vi "LCP table array ans.vi"(6 "LSP Table":string[][](table) caption="LS Table", 8 "error in (no error)":errorcluster caption="error in", 9 "LAP Table":string[][](table), 10 "LCP Table":string[][](table) caption="CP Table", 11 "Tag cluster_B":T3) -> (0 "error out":errorcluster, 1 "LSPX_C2":T4, 2 "LSPX_C1":T5, 3 "LCPX_C1":T6, 5 "LCPX_CZ":T1)   [LabVIEW 2018]
panel:
  out "LCPX_C2":T2
  out "LA_Signal Intensity [pA]":dbl[](array[numeric])
  out "MS_IDX":i32[](array[numeric])
  out "LA_Time":dbl[](array[numeric])
  out "LA_Relative Averaged Data":dbl[](array[numeric])
  out "LAP Table Tag":string[](array[string])
  out "Signal Intensity [pA]":dbl[](array[numeric])
  out "Base Number":i32[](array[numeric])
  out "L#":i32[](array[numeric])
  out "Signal Intensity [pA]":string[](array[string])
  out "Base Number":string[](array[string])
  out "Mx Right Read Seq":string[](array[string])
  out "L#":string[](array[string])
  out "Assinged Sequence":string[](array[string])
  out "Signal End [s]":dbl[](array[numeric])
  out "Signal Start [s]":dbl[](array[numeric])
  out "S IDX":i32[](array[numeric])
  out "Mx Right No":i32[](array[numeric])
  out "Seq ENo":i32[](array[numeric])
  out "Seq SNo":i32[](array[numeric])
  out "Signal End [s]":string[](array[string])
  out "S IDX":string[](array[string])
  out "Signal Start [s]":string[](array[string])
  out "Direction":string[](array[string])
  out "Seq ENo":string[](array[string])
  out "Mx Right No":string[](array[string])
  out "Seq SNo":string[](array[string])
  out "5’→3'":bool[](array[boolean])
  out "5’→3'":dbl
  out "Signal Length [ms]":dbl[](array[numeric])
  out "Q value [x]":dbl[](array[numeric])
  out "Signal Intensity [pA]":dbl[](array[numeric])
  out "AS IDX":i32[](array[numeric])
  out "Time":dbl[](array[numeric])
  out "Relative Averaged Data":dbl[](array[numeric])
  out "LCP Table Tag":string[](array[string])
  out "LSP Table Tag":string[](array[string])
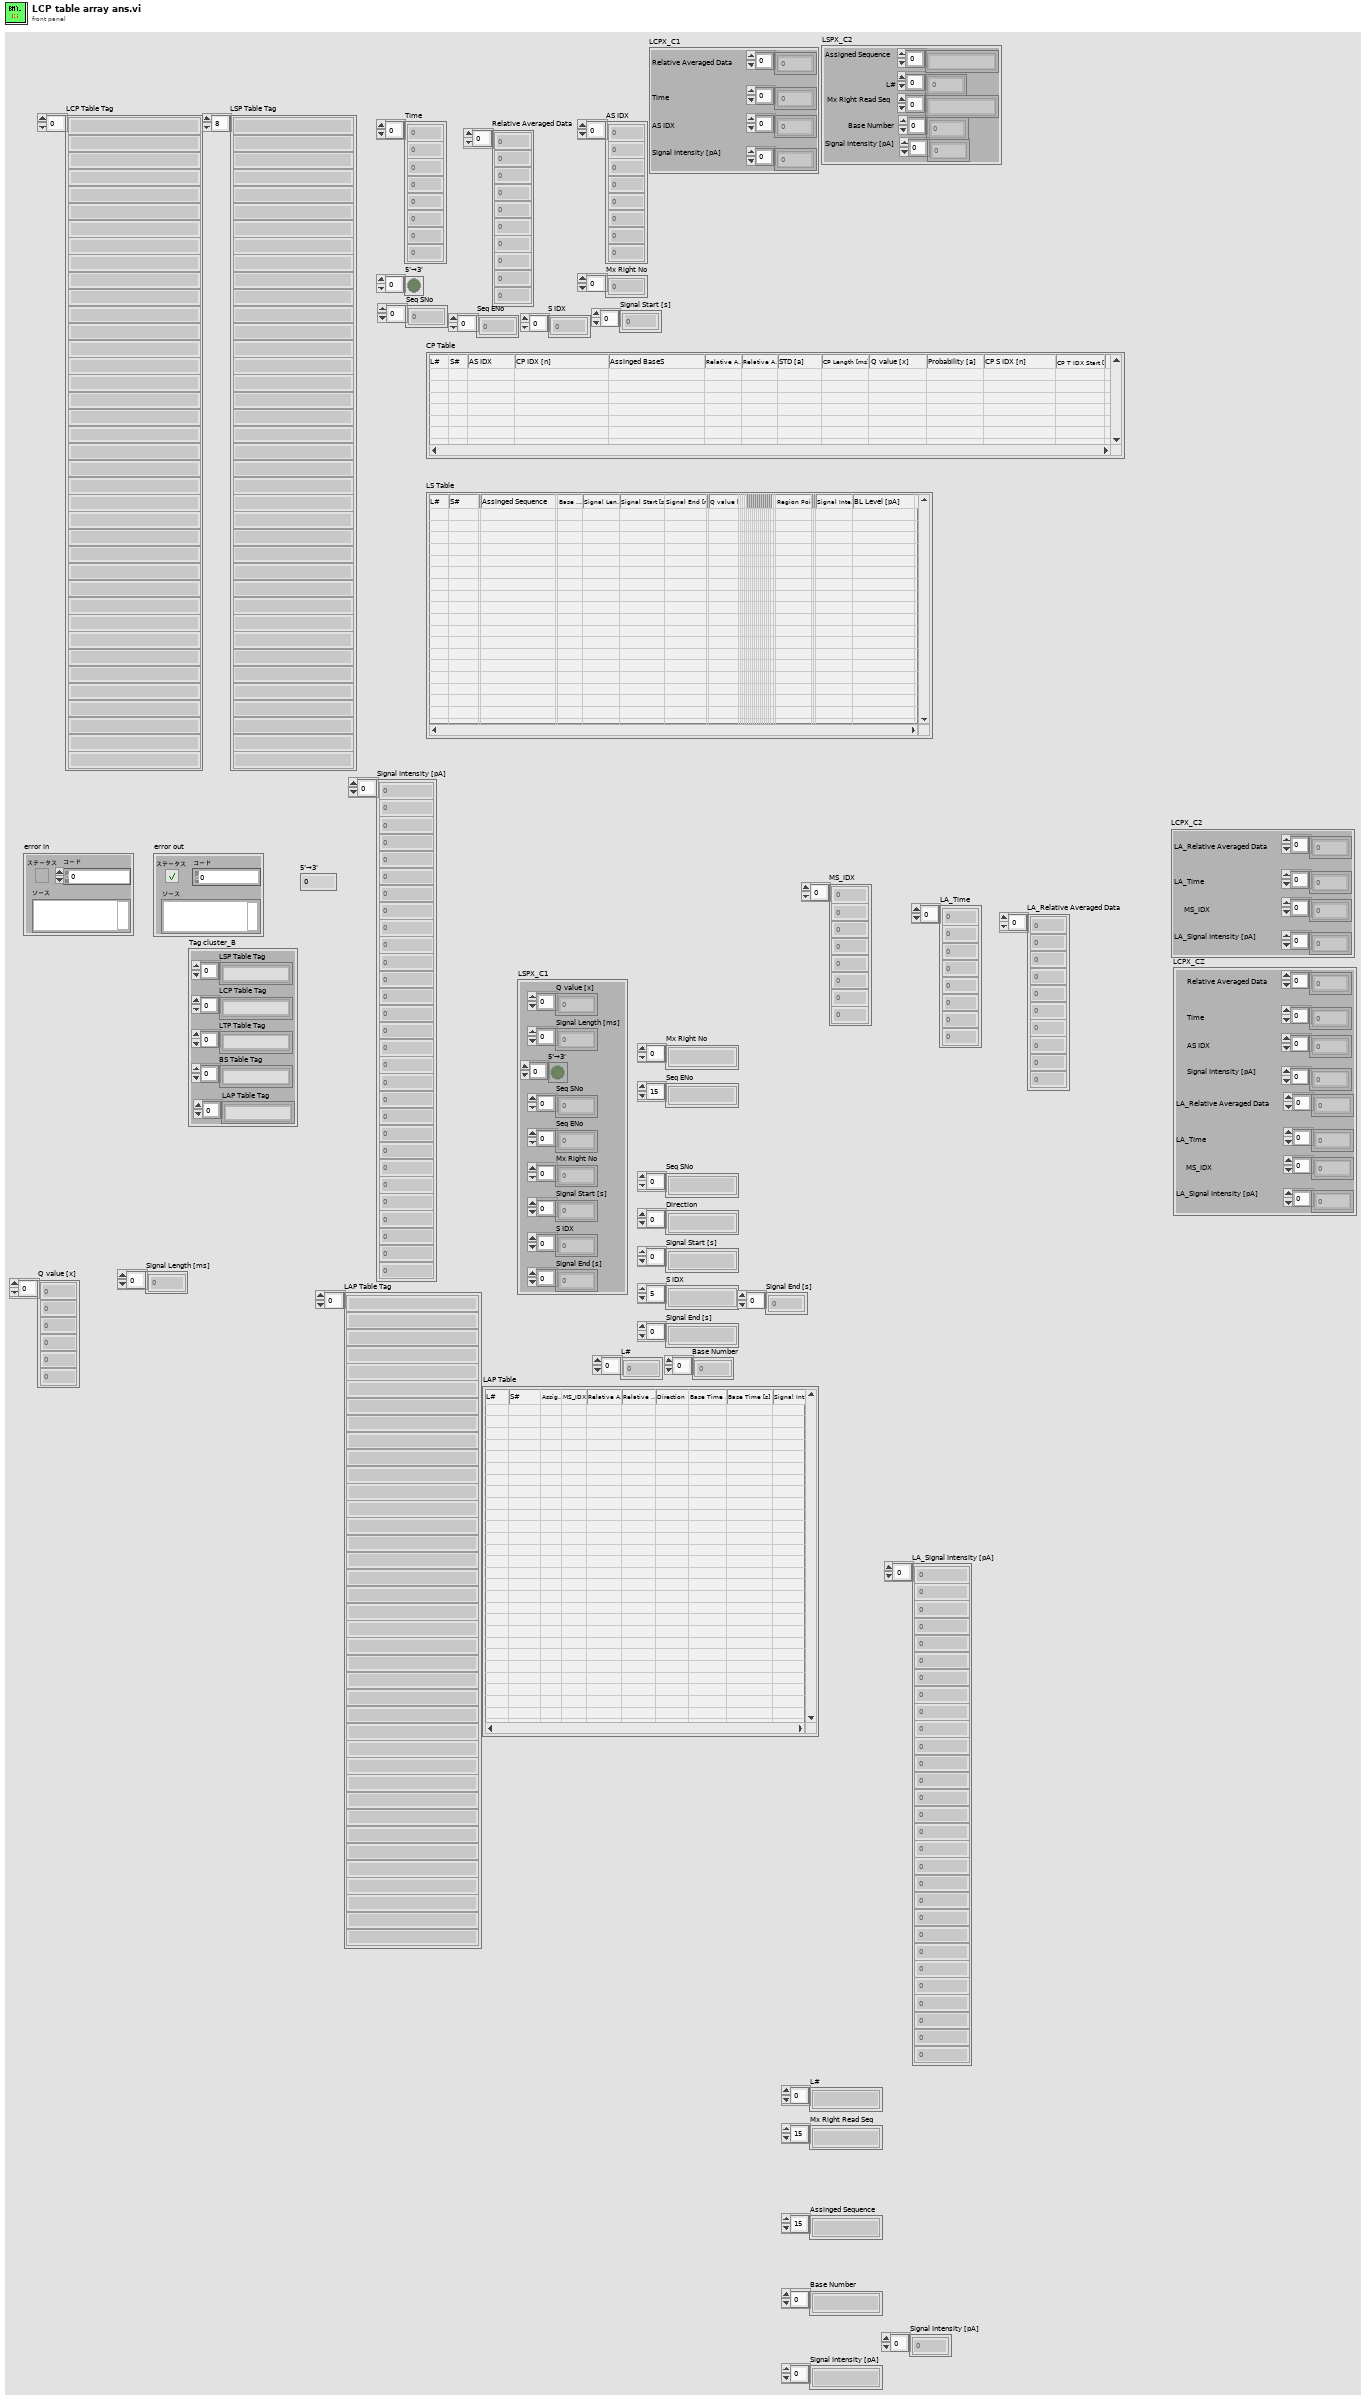
[diagram p1: front panel]
types:
  T1 = cluster{"Relative Averaged Data":dbl[], "Time":dbl[], "AS IDX":i32[], "Signal Intensity [pA]":dbl[], "LA_Relative Averaged Data":dbl[], "LA_Time":dbl[], "MS_IDX":i32[], "LA_Signal Intensity [pA]":dbl[]}
  T2 = cluster{"LA_Relative Averaged Data":dbl[], "LA_Time":dbl[], "MS_IDX":i32[], "LA_Signal Intensity [pA]":dbl[]}
  T3 = cluster{"LSP Table Tag":string[], "LCP Table Tag":string[], "LTP Table Tag":string[], "BS Table Tag":string[], "LAP Table Tag":string[]}
  T4 = cluster{"Assigned Sequence":string[], "L#":i32[], "Mx Right Read Seq":string[], "Base Number":i32[], "Signal Intensity [pA]":dbl[]}
  T5 = cluster{"Q value [x]":dbl[], "Signal Length [ms]":dbl[], "5’→3'":bool[], "Seq SNo":i32[], "Seq ENo":i32[], "Mx Right No":i32[], "Signal Start [s]":dbl[], "S IDX":i32[], "Signal End [s]":dbl[]}
  T6 = cluster{"Relative Averaged Data":dbl[], "Time":dbl[], "AS IDX":i32[], "Signal Intensity [pA]":dbl[]}
  T7 = cluster{dbl[], dbl[], i32[], dbl[], dbl[], dbl[], i32[], dbl[]}
  T8 = cluster{dbl[], dbl[], bool[], i32[], i32[], i32[], dbl[], i32[], dbl[]}
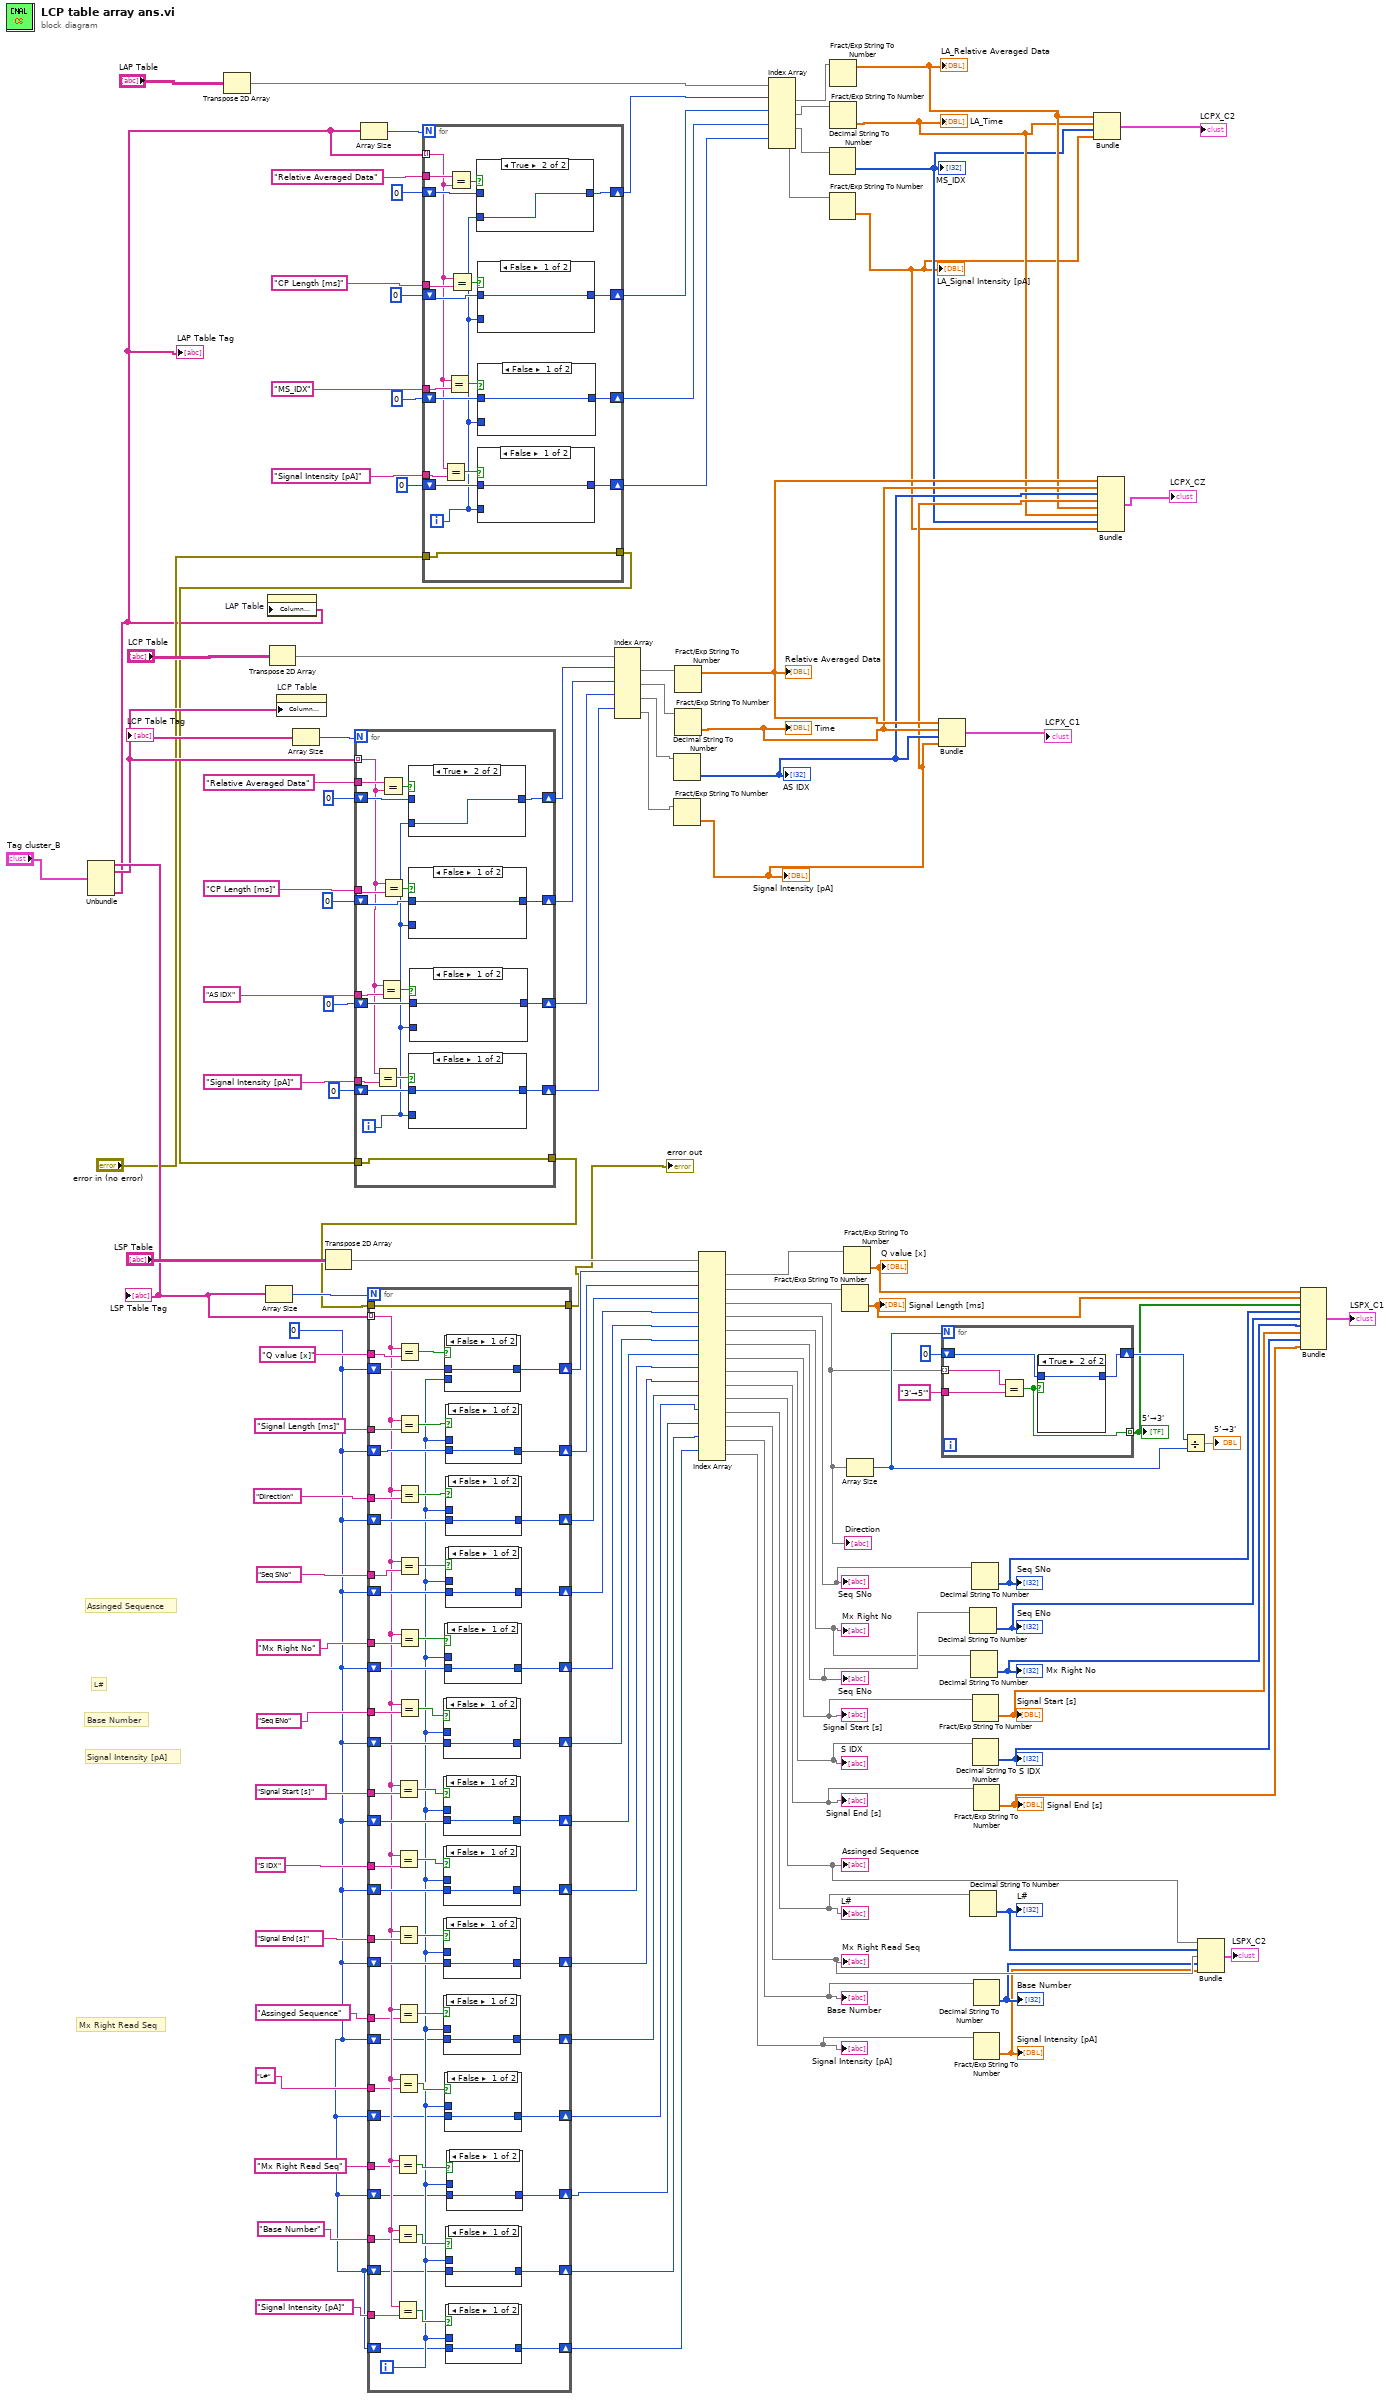
[diagram p0: block diagram]
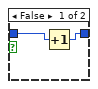
[diagram p6: hidden frame]
diagram:
  w55 = 0
  # "Mx Right Read Seq"
  # "Signal Intensity [pA]"
  # "Base Number"
  # "Assinged Sequence"
  # "L#"
  n1 = Unbundle("Tag cluster_B") -> ("LSP Table Tag"=w34:string[], "LCP Table Tag"=w33:string[], "LAP Table Tag"=w15:string[])  [unwired: 2 out]
  "LSP Table Tag" <- w34
  "LCP Table Tag" <- w33
  "LAP Table Tag" <- w15
  n2 = Transpose 2D Array(2D array="LAP Table") -> (transposed array=w20:string[][])
  n3 = Array Size(array=w34) -> (size(s)=w106:i32)
  n4 = property on="LAP Table" class="Tbl (strict)"("Column Headers[]"=w15) -> ()  [unwired: 2 in, 2 out]
  n5 = Transpose 2D Array(2D array="LCP Table") -> (transposed array=w113:string[][])
  n6 = property on="LCP Table" class="Tbl (strict)"("Column Headers[]"=w33) -> ()  [unwired: 2 in, 2 out]
  n7 = Array Size(array=w33) -> (size(s)=w108:i32)
  n8 = Transpose 2D Array(2D array="LSP Table") -> (transposed array=w101:string[][])
  n9 = Array Size(array=w15) -> (size(s)=w24:i32)
  n10 = for {
    N: w24 -> [_]
    tunnel: "Relative Averaged Data" -> [w141]
    tunnel: w15 -> [w126] mode=indexing
    shift-right: [w139] -> w19
    shift-left: 0 -> [w138]
    tunnel: "CP Length [ms]" -> [w137]
    shift-right: [w135] -> w18
    shift-left: 0 -> [w134]
    shift-right: [w132] -> w17
    shift-left: 0 -> [w131]
    tunnel: "MS_IDX" -> [w130]
    shift-right: [w129] -> w16
    shift-left: 0 -> [w128]
    tunnel: "Signal Intensity [pA]" -> [w125]
    tunnel: "error in (no error)" -> [w124]
    tunnel: [w124] -> w22
    i -> [w123]
    n11 = Equal?(x=w126, y=w125) -> (x = y?=w127:bool)
    n12 = Equal?(x=w126, y=w130) -> (x = y?=w133:bool)
    n13 = Equal?(x=w141, y=w126) -> (x = y?=w140:bool)
    n14 = Equal?(x=w126, y=w137) -> (x = y?=w136:bool)
    n15 = case shown="True" w140 {
      tunnel: w123 -> [_ w149]
      tunnel: [w148 w149] -> w139
      tunnel: w138 -> [w148 _]
      frame False {
      }
      frame True {
      }
    }
    n16 = case shown="False" w136 {
      tunnel: w123 -> [_ w147]
      tunnel: [w146 w147] -> w135
      tunnel: w134 -> [w146 _]
      frame False {
      }
      frame True {
      }
    }
    n17 = case shown="False" w127 {
      tunnel: w123 -> [_ w143]
      tunnel: [w142 w143] -> w129
      tunnel: w128 -> [w142 _]
      frame False {
      }
      frame True {
      }
    }
    n18 = case shown="False" w133 {
      tunnel: w123 -> [_ w145]
      tunnel: [w144 w145] -> w132
      tunnel: w131 -> [w144 _]
      frame False {
      }
      frame True {
      }
    }
  }
  n19 = for {
    N: w108 -> [_]
    tunnel: "Relative Averaged Data" -> [w168]
    tunnel: w33 -> [w153] mode=indexing
    shift-right: [w166] -> w39
    shift-left: 0 -> [w165]
    tunnel: "CP Length [ms]" -> [w164]
    shift-right: [w162] -> w38
    shift-left: 0 -> [w161]
    shift-right: [w159] -> w110
    shift-left: 0 -> [w158]
    tunnel: "AS IDX" -> [w157]
    shift-right: [w156] -> w37
    shift-left: 0 -> [w155]
    tunnel: "Signal Intensity [pA]" -> [w152]
    tunnel: w22 -> [w151]
    tunnel: [w151] -> w62
    i -> [w150]
    n20 = Equal?(x=w153, y=w152) -> (x = y?=w154:bool)
    n21 = Equal?(x=w153, y=w157) -> (x = y?=w160:bool)
    n22 = Equal?(x=w168, y=w153) -> (x = y?=w167:bool)
    n23 = Equal?(x=w153, y=w164) -> (x = y?=w163:bool)
    n24 = case shown="True" w167 {
      tunnel: w150 -> [_ w176]
      tunnel: [w175 w176] -> w166
      tunnel: w165 -> [w175 _]
      frame False {
      }
      frame True {
      }
    }
    n25 = case shown="False" w163 {
      tunnel: w150 -> [_ w174]
      tunnel: [w173 w174] -> w162
      tunnel: w161 -> [w173 _]
      frame False {
      }
      frame True {
      }
    }
    n26 = case shown="False" w154 {
      tunnel: w150 -> [_ w170]
      tunnel: [w169 w170] -> w156
      tunnel: w155 -> [w169 _]
      frame False {
      }
      frame True {
      }
    }
    n27 = case shown="False" w160 {
      tunnel: w150 -> [_ w172]
      tunnel: [w171 w172] -> w159
      tunnel: w158 -> [w171 _]
      frame False {
      }
      frame True {
      }
    }
  }
  n28 = for {
    N: w106 -> [_]
    tunnel: w34 -> [w198] mode=indexing
    tunnel: "Q value [x]" -> [w235]
    tunnel: "Signal Length [ms]" -> [w234]
    tunnel: "Direction" -> [w233]
    shift-right: [w229] -> w102
    shift-left: w55 -> [w228]
    shift-right: [w227] -> w99
    shift-left: w55 -> [w226]
    shift-right: [w225] -> w97
    shift-left: w55 -> [w224]
    tunnel: "Seq SNo" -> [w223]
    tunnel: "Mx Right No" -> [w222]
    tunnel: "Seq ENo" -> [w221]
    tunnel: "Signal Start [s]" -> [w220]
    tunnel: "S IDX" -> [w219]
    tunnel: "Signal End [s]" -> [w218]
    shift-right: [w211] -> w84
    shift-left: w55 -> [w210]
    shift-right: [w209] -> w83
    shift-left: w55 -> [w208]
    shift-right: [w207] -> w82
    shift-left: w55 -> [w206]
    shift-right: [w205] -> w80
    shift-left: w55 -> [w204]
    shift-right: [w203] -> w79
    shift-left: w55 -> [w202]
    shift-right: [w201] -> w78
    shift-left: w55 -> [w200]
    tunnel: w62 -> [w199]
    tunnel: [w199] -> w61
    tunnel: "Base Number" -> [w197]
    tunnel: "Signal Intensity [pA]" -> [w192]
    tunnel: "Assinged Sequence" -> [w190]
    tunnel: "L#" -> [w189]
    shift-right: [w188] -> w54
    shift-left: w55 -> [w186]
    shift-right: [w185] -> w53
    shift-left: w55 -> [w184]
    shift-right: [w183] -> w51
    shift-left: w55 -> [w182]
    shift-right: [w181] -> w50
    shift-left: w55 -> [w180]
    shift-right: [w179] -> w49
    shift-left: w55 -> [w178]
    tunnel: "Mx Right Read Seq" -> [w177]
    i -> [w187]
    n29 = Equal?(x=w198, y=w177) -> (x = y?=w194:bool)
    n30 = Equal?(x=w198, y=w197) -> (x = y?=w193:bool)
    n31 = Equal?(x=w198, y=w192) -> (x = y?=w191:bool)
    n32 = Equal?(x=w198, y=w220) -> (x = y?=w214:bool)
    n33 = Equal?(x=w198, y=w219) -> (x = y?=w213:bool)
    n34 = Equal?(x=w198, y=w218) -> (x = y?=w212:bool)
    n35 = Equal?(x=w198, y=w190) -> (x = y?=w196:bool)
    n36 = Equal?(x=w198, y=w189) -> (x = y?=w195:bool)
    n37 = Equal?(x=w198, y=w235) -> (x = y?=w232:bool)
    n38 = Equal?(x=w198, y=w234) -> (x = y?=w231:bool)
    n39 = Equal?(x=w198, y=w233) -> (x = y?=w230:bool)
    n40 = Equal?(x=w198, y=w223) -> (x = y?=w217:bool)
    n41 = Equal?(x=w198, y=w222) -> (x = y?=w216:bool)
    n42 = Equal?(x=w198, y=w221) -> (x = y?=w215:bool)
    n43 = case shown="False" w215 {
      tunnel: w187 -> [_ w253]
      tunnel: [w252 w253] -> w207
      tunnel: w206 -> [w252 _]
      frame False {
      }
      frame True {
      }
    }
    n44 = case shown="False" w214 {
      tunnel: w187 -> [_ w251]
      tunnel: [w250 w251] -> w205
      tunnel: w204 -> [w250 _]
      frame False {
      }
      frame True {
      }
    }
    n45 = case shown="False" w213 {
      tunnel: w187 -> [_ w249]
      tunnel: [w248 w249] -> w203
      tunnel: w202 -> [w248 _]
      frame False {
      }
      frame True {
      }
    }
    n46 = case shown="False" w212 {
      tunnel: w187 -> [_ w247]
      tunnel: [w246 w247] -> w201
      tunnel: w200 -> [w246 _]
      frame False {
      }
      frame True {
      }
    }
    n47 = case shown="False" w196 {
      tunnel: w187 -> [_ w245]
      tunnel: [w244 w245] -> w188
      tunnel: w186 -> [w244 _]
      frame False {
      }
      frame True {
      }
    }
    n48 = case shown="False" w232 {
      tunnel: w187 -> [_ w263]
      tunnel: [w262 w263] -> w229
      tunnel: w228 -> [w262 _]
      frame False {
      }
      frame True {
      }
    }
    n49 = case shown="False" w216 {
      tunnel: w187 -> [_ w255]
      tunnel: [w254 w255] -> w209
      tunnel: w208 -> [w254 _]
      frame False {
      }
      frame True {
      }
    }
    n50 = case shown="False" w195 {
      tunnel: w187 -> [_ w243]
      tunnel: [w242 w243] -> w185
      tunnel: w184 -> [w242 _]
      frame False {
      }
      frame True {
      }
    }
    n51 = case shown="False" w231 {
      tunnel: w187 -> [_ w261]
      tunnel: [w260 w261] -> w227
      tunnel: w226 -> [w260 _]
      frame False {
      }
      frame True {
      }
    }
    n52 = case shown="False" w230 {
      tunnel: w187 -> [_ w259]
      tunnel: [w258 w259] -> w225
      tunnel: w224 -> [w258 _]
      frame False {
      }
      frame True {
      }
    }
    n53 = case shown="False" w217 {
      tunnel: w187 -> [_ w257]
      tunnel: [w256 w257] -> w211
      tunnel: w210 -> [w256 _]
      frame False {
      }
      frame True {
      }
    }
    n54 = case shown="False" w193 {
      tunnel: w187 -> [_ w239]
      tunnel: [w238 w239] -> w181
      tunnel: w180 -> [w238 _]
      frame False {
      }
      frame True {
      }
    }
    n55 = case shown="False" w191 {
      tunnel: w187 -> [_ w237]
      tunnel: [w236 w237] -> w179
      tunnel: w178 -> [w236 _]
      frame False {
      }
      frame True {
      }
    }
    n56 = case shown="False" w194 {
      tunnel: w187 -> [_ w241]
      tunnel: [w240 w241] -> w183
      tunnel: w182 -> [w240 _]
      frame False {
      }
      frame True {
      }
    }
  }
  "error out" <- w61
  n57 = Index Array(array=w113, index (row) #1=w39, index (row) #2=w38, index (row) #3=w110, index (row) #4=w37) -> (element #1=w112:string[], element #2=w111:string[], element #3=w109:string[], element #4=w107:string[])  [unwired: 4 in]
  n58 = Decimal String To Number(string=w109) -> (number=w7:i32[])  [unwired: 2 in, 1 out]
  "AS IDX" <- w7
  n59 = Fract/Exp String To Number(string=w107) -> (number=w6:dbl[])  [unwired: 3 in, 1 out]
  "Signal Intensity [pA]" <- w6
  n60 = Fract/Exp String To Number(string=w112) -> (number=w9:dbl[])  [unwired: 3 in, 1 out]
  "Relative Averaged Data" <- w9
  n61 = Fract/Exp String To Number(string=w111) -> (number=w8:dbl[])  [unwired: 3 in, 1 out]
  "Time" <- w8
  n62 = Index Array(array=w101, index (row) #1=w102, index (row) #2=w99, index (row) #3=w97, index (row) #4=w84, index (row) #5=w83, index (row) #6=w82, index (row) #7=w80, index (row) #8=w79, index (row) #9=w78, index (row) #10=w54, index (row) #11=w53, index (row) #12=w51, index (row) #13=w50, index (row) #14=w49) -> (element #1=w100:string[], element #2=w98:string[], element #3=w81:string[], element #4=w77:string[], element #5=w75:string[], element #6=w76:string[], element #7=w74:string[], element #8=w73:string[], element #9=w72:string[], element #10=w45:string[], element #11=w48:string[], element #12=w43:string[], element #13=w47:string[], element #14=w46:string[])  [unwired: 14 in]
  "Seq SNo" <- w77
  "Mx Right No" <- w75
  "Seq ENo" <- w76
  "Direction" <- w81
  "Signal Start [s]" <- w74
  "S IDX" <- w73
  "Signal End [s]" <- w72
  "Assinged Sequence" <- w45
  "L#" <- w48
  "Mx Right Read Seq" <- w43
  "Base Number" <- w47
  "Signal Intensity [pA]" <- w46
  n63 = Index Array(array=w20, index (row) #1=w19, index (row) #2=w18, index (row) #3=w17, index (row) #4=w16) -> (element #1=w13:string[], element #2=w12:string[], element #3=w11:string[], element #4=w10:string[])  [unwired: 4 in]
  n64 = Decimal String To Number(string=w11) -> (number=w3:i32[])  [unwired: 2 in, 1 out]
  "MS_IDX" <- w3
  n65 = Fract/Exp String To Number(string=w10) -> (number=w2:dbl[])  [unwired: 3 in, 1 out]
  "LA_Signal Intensity [pA]" <- w2
  n66 = Fract/Exp String To Number(string=w13) -> (number=w5:dbl[])  [unwired: 3 in, 1 out]
  "LA_Relative Averaged Data" <- w5
  n67 = Fract/Exp String To Number(string=w12) -> (number=w4:dbl[])  [unwired: 3 in, 1 out]
  "LA_Time" <- w4
  n68 = Fract/Exp String To Number(string=w98) -> (number=w70:dbl[])  [unwired: 3 in, 1 out]
  "Signal Length [ms]" <- w70
  n69 = Fract/Exp String To Number(string=w100) -> (number=w71:dbl[])  [unwired: 3 in, 1 out]
  "Q value [x]" <- w71
  n70 = Array Size(array=w81) -> (size(s)=w91:i32)
  n71 = Bundle(w9, w8, w7, w6) -> (→"LCPX_C1":cluster{dbl[], dbl[], i32[], dbl[]})  [unwired: 1 in]
  n72 = for {
    N: w91 -> [_]
    tunnel: w81 -> [w268] mode=indexing
    tunnel: "3'→5'" -> [w267]
    tunnel: [w266] -> w69 mode=indexing
    shift-right: [w265] -> w94
    shift-left: 0 -> [w264]
    n73 = Equal?(x=w268, y=w267) -> (x = y?=w266:bool)
    n74 = case shown="True" w266 {
      tunnel: [w269 w271] -> w265
      tunnel: w264 -> [w270 w271]
      frame False {
        n75 = Increment(x=w270) -> (x+1=w269:i32)
      }
      frame True {
      }
    }
  }
  "5’→3'" <- w69
  n76 = Decimal String To Number(string=w76) -> (number=w67:i32[])  [unwired: 2 in, 1 out]
  "Seq ENo" <- w67
  n77 = Decimal String To Number(string=w48) -> (number=w44:i32[])  [unwired: 2 in, 1 out]
  "L#" <- w44
  n78 = Decimal String To Number(string=w75) -> (number=w66:i32[])  [unwired: 2 in, 1 out]
  "Mx Right No" <- w66
  n79 = Decimal String To Number(string=w77) -> (number=w68:i32[])  [unwired: 2 in, 1 out]
  "Seq SNo" <- w68
  n80 = Fract/Exp String To Number(string=w74) -> (number=w65:dbl[])  [unwired: 3 in, 1 out]
  "Signal Start [s]" <- w65
  n81 = Decimal String To Number(string=w73) -> (number=w64:i32[])  [unwired: 2 in, 1 out]
  "S IDX" <- w64
  n82 = Fract/Exp String To Number(string=w72) -> (number=w63:dbl[])  [unwired: 3 in, 1 out]
  "Signal End [s]" <- w63
  n83 = Decimal String To Number(string=w47) -> (number=w42:i32[])  [unwired: 2 in, 1 out]
  "Base Number" <- w42
  n84 = Fract/Exp String To Number(string=w46) -> (number=w41:dbl[])  [unwired: 3 in, 1 out]
  "Signal Intensity [pA]" <- w41
  n85 = Bundle(w5, w4, w3, w2) -> (→"LCPX_C2":cluster{dbl[], dbl[], i32[], dbl[]})  [unwired: 1 in]
  n86 = Bundle(w9, w8, w7, w6, w5, w4, w3, w2) -> (→"LCPX_CZ":T7)  [unwired: 1 in]
  n87 = Divide(x=w94, y=w91) -> (x/y=→"5’→3'":dbl)
  n88 = Bundle(w45, w44, w43, w42, w41) -> (→"LSPX_C2":cluster{string[], i32[], string[], i32[], dbl[]})  [unwired: 1 in]
  n89 = Bundle(w71, w70, w69, w68, w67, w66, w65, w64, w63) -> (→"LSPX_C1":T8)  [unwired: 1 in]
